vi "test--#FF7FFF.vi"(11 "Test Case In":refnum<class "HSL Integer Rounding.lvclass">) -> (0 "error out":errorcluster, 3 "Test Case Out":refnum<class "HSL Integer Rounding.lvclass">)   [LabVIEW 2021, in "HSL Integer Rounding.lvclass"]
uses:
  HSL Integer Rounding.lvclass
  C:/Program Files/National Instruments/LabVIEW 2026/vi.lib/Astemes/LUnit/Test Case.lvclass
  <vilib>/Astemes/LUnit/Test Case.lvclass/Test Case.ctl
  4993e8ee-a06a-463a-9684-69129f64d5ce.vi
  src/Material SubVIs/tsc--RGB to Color.vi
  <vilib>/Astemes/LUnit/Core/LUnit Test Case/Private/Append Pass Result.vi
  <vilib>/Astemes/LUnit/Core/LUnit Test Case/Private/Append Fail Result.vi
  4993e8ee-a06a-463a-9684-69129f64d5ce.vi/9c5d11cd-9439-4240-a1ee-d9baace9c924.vi
  <vilib>/Astemes/LUnit/Core/LUnit Test Case/Private/Run In UI.vi
  <vilib>/Utility/error.llb/Clear Errors.vi
  <vilib>/Utility/colorconv.llb/Color to RGB.vi
  src/Material SubVIs/Material SubVIs.lvlib
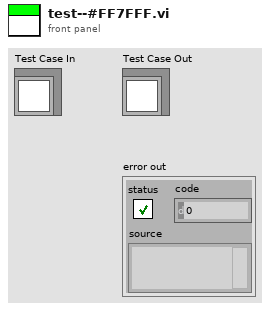
[diagram p1: front panel]
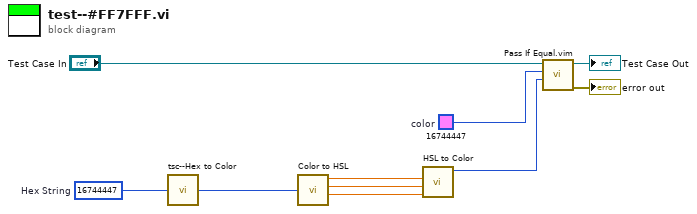
[diagram p0: block diagram]
diagram:
  w2 = u32 16744447  # color
  w3 = u32 16744447  # Hex String
  n1 = call "tsc--Hex to Color.vi"("Hex String"=w3) -> ("Color"=w7:u32)  [unwired: 4 in]
  n2 = call "Color to HSL.vi"("Color In"=w7) -> ("H (degrees)"=w6:dbl, "S (%)"=w5:dbl, "L (%)"=w4:dbl)  [unwired: 4 in, 1 out]
  n3 = call "HSL to Color.vi"("L (%)"=w4, "S (%)"=w5, "H (degrees)"=w6) -> ("Color out"=w1:u32)  [unwired: 5 in, 3 out]
  n4 = call "Pass If Equal.vim"("Actual"=w1, "Expected"=w2, "LUnit Test Case In"="Test Case In") -> ("error out"=→"error out":errorcluster, "LUnit Test Case Out"=→"Test Case Out":refnum<class "HSL Integer Rounding.lvclass">)  [unwired: 7 in]
